vi "Stop Core.vi"(10 "final error code":i32, 11 "HamamatsuFluor in":refnum<class "HamamatsuFluor.lvclass">) -> (3 "HamamatsuFluor out":refnum<class "HamamatsuFluor.lvclass">)   [LabVIEW 2020, in "DAQ Timed SPIM.lvlib" / "HamamatsuFluor_v2.lvlib" / "HamamatsuFluor.lvclass"]
doc: "(<B>Filename</B>: Actor Framework.lvlib:Actor.lvclass:Stop Core.vi)\n\nDefines what the actor does before it stops. Use the <B>final error code</B> input to determine whether the actor shut down in response to an error.\n\nBy default, this method passes the Stop message along to all auto-stop nested actors. A descendant class may override this method to define additional behavior, such as shutting down any processes the actor initiated in its override of the Actor Core method."
uses:
  HamamatsuFluor.lvclass
  HamamatsuFluor.lvclass/HamamatsuFluor.ctl
  <vilib>/Utility/error.llb/Error Cluster From Error Code.vi
  Abstract DAQ Triggered Actor/Abstract DAQ Triggered Actor.lvclass
  WIN Memory Map.llb/WIN MMAP.lvlib
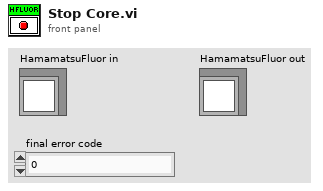
[diagram p1: front panel]
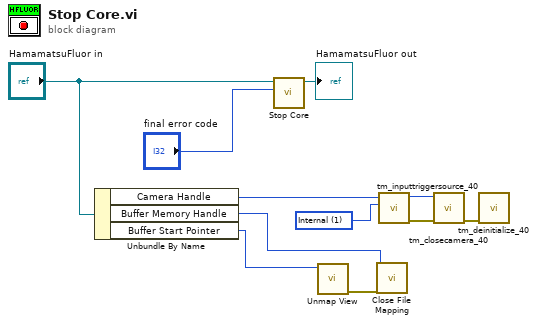
[diagram p0: block diagram]
diagram:
  w8 = 1 items=["Internal"=1, "External"=2, "Software"=3, "Master Pulse"=4] ("Source")
  n1 = Unbundle By Name("HamamatsuFluor in") -> ("Camera Handle"=w5:u32, "Buffer Memory Handle"=w3:u64, "Buffer Start Pointer"=w1:u64)
  n2 = call-parent "Stop Core.vi"("final error code"="final error code", "Actor in"="HamamatsuFluor in") -> ("Actor out"=→"HamamatsuFluor out":refnum<class "HamamatsuFluor.lvclass">)  [unwired: 9 in]
  n3 = call "Unmap View.vi"("start address"=w1) -> ("error out"=w2:errorcluster)  [unwired: 10 in]
  n4 = call "Close File Mapping.vi"("error in (no error)"=w2, "handle"=w3) -> ()  [unwired: 9 in, 1 out]
  n5 = call <userlib>:"tm_inputtriggersource_40.vi"("Source"=w8, "Handle in"=w5) -> ("error out"=w7:errorcluster, "Handle out"=w6:u32)  [unwired: 8 in]
  n6 = call <userlib>:"tm_closecamera_40.vi"("error in (no error)"=w7, "Handle in"=w6) -> ("error out"=w9:errorcluster)  [unwired: 9 in]
  n7 = call <userlib>:"tm_deinitialize_40.vi"("error in (no error)"=w9) -> ()  [unwired: 10 in, 1 out]
